vi "Common_UpdateAttributes.vi"(1 "ClassPath/LvClassRef":variant, 2 "NewAttributes":string, 3 "ClassInfo":T4[](array[typedef]), 5 "error in (no error)":errorcluster, 6 "Don't Prompt (False)":bool, 7 "Attributes":T1[](array[typedef]), 8 "Stereotype":string, 9 "Ctl-Description":string) -> (15 "CtlPath":path, 18 "Cancel":bool, 19 "error out":errorcluster)   [LabVIEW 2020] (continued)
 terminals)", "Swap Bytes", "Swap Values", "Swap Vector Element", "Swap Words", "Tab Constant", "Tab Control (classic)", "Tab Control (modern)", "Tab Control (NXG Style)", "Tab Control (system)", "Table (classic)", "Table (modern)", "Table (system)", "Tag Attribute Ring", "Tangent", "Tank (classic)", "Tank (modern)", "Target Structure", "TCP Close Connection", "TCP Create Listener", "TCP Flattened Read", "TCP Flattened Write", "TCP Flex Read", "TCP Flex Write", "TCP Network Connection Refnum", "TCP Open Connection", "TCP Read", "TCP Wait On Listener", "TCP Write", "TDMS Advanced Asynchronous Read (Data Ref)", "TDMS Advanced Asynchronous Write (Data Ref)", "TDMS Close", "TDMS Configure Asynchronous Reads (Data Ref)", "TDMS Configure Asynchronous Writes (Data Ref)", "TDMS Defragment", "TDMS Delete Data", "TDMS File", "TDMS Flush", "TDMS Get Asynchronous Read Status (Data Ref)", "TDMS Get Asynchronous Write Status (Data Ref)", "TDMS Get Properties", "TDMS In Memory Close", "TDMS In Memory Open", "TDMS In Memory Read Bytes", "TDMS List Contents", "TDMS Open", "TDMS Read", "TDMS Refnum To File ID", "TDMS Set Properties", "TDMS Write", "TDMS Write IP", "Temporary Directory", "TestSRQ", "TestSys", "Text & Pict Ring (classic)", "Text & Pict Ring (modern)", "Text Button", "Text Ring (block diagram constant)", "Text Ring (classic)", "Text Ring (modern)", "Text Ring (system)", "Text to UTF-8", "Thermometer (classic)", "Thermometer (modern)", "Threshold 1D Array", "Tick Count (ms)", "Time Stamp (block diagram constant)", "Time Stamp Control (classic)", "Time Stamp Control (modern)", "Time Stamp Control (system)", "Time Stamp Indicator (classic)", "Time Stamp Indicator (modern)", "Timed Loop", "Timed Sequence", "TLS configuration", "TLS Connection?", "To Byte Integer", "To Double Precision Complex", "To Double Precision Float", "To Extended Precision Complex", "To Extended Precision Float", "To Fixed-Point", "To Long Integer", "To Lower Case", "To More Generic Class", "To More Specific Class", "To OLE Variant", "To Probe String", "To Quad Integer", "To Single Precision Complex", "To Single Precision Float", "To Time Stamp", "To Unsigned Byte Integer", "To Unsigned Long Integer", "To Unsigned Quad Integer", "To Unsigned Word Integer", "To Upper Case", "To Variant", "To Word Integer", "Traditional DAQ Channel (block diagram constant)", "Traditional DAQ Channel (classic)", "Traditional DAQ Channel (modern)", "Transpose 1D Array", "Transpose 2D Array", "Transpose Matrix", "Tree (classic)", "Tree (modern)", "Tree (system)", "Trigger", "TriggerList", "Two Button Dialog", "Type and Creator", "Type Cast", "Type Error", "Type Must Be Array", "Type Must Be Cluster", "Type Of", "Type Specialization Structure", "UDP Close", "UDP Multicast Open", "UDP Network Connection Refnum", "UDP Open", "UDP Read", "UDP Write", "Unbitpack from Array", "Unbundle", "Unbundle By Name", "Unflatten From JSON", "Unflatten From String", "Unflatten From XML", "Unleak Variant Value Reference", "Unpackage Matrix", "Unregister For Events", "Unregister Session", "Up Arrow", "Up Bow Valve (flat)", "Up Bow Valve (outline)", "Up Bow Valve (shaded)", "Up Rect Valve (flat)", "Up Rect Valve (outline)", "Up Rect Valve (shaded)", "Up Tee (flat)", "Up Tee (shaded)", "User Defined Refnum", "User Defined Refnum Tag (block diagram constant)", "User Defined Refnum Tag (classic)", "User Defined Refnum Tag (modern)", "User Defined Refnum Tag Flatten (classic)", "User Defined Refnum Tag Flatten (modern)", "User Defined Tag (block diagram constant)", "User Defined Tag (classic)", "User Defined Tag (modern)", "User Item", "UTF-8 String To Byte Array", "UTF-8 to Text", "Variable Class Specifier Constant", "Variable Name Constant", "Variant", "Variant To Data", "Variant To Flattened String", "Vert Line", "Vert Pipe (flat)", "Vert Pipe (shaded)", "Vert Rocker", "Vertical Fill Slide (classic)", "Vertical Fill Slide (modern)", "Vertical Gradient Oval", "Vertical Gradient Rectangle", "Vertical Gradient Rounded Rectangle", "Vertical Graduated Bar", "Vertical Pointer Slide (classic)", "Vertical Pointer Slide (modern)", "Vertical Pointer Slide (system)", "Vertical Progress Bar (modern)", "Vertical Progress Bar (system)", "Vertical Scrollbar", "Vertical Slide (system)", "Vertical Slide Switch (classic)", "Vertical Slide Switch (modern)", "Vertical Smooth Box", "Vertical Splitter Bar", "Vertical Splitter Bar (Classic)", "Vertical Splitter Bar (NXG Style)", "Vertical Splitter Bar (System)", "Vertical Switch", "Vertical Toggle Switch (classic)", "Vertical Toggle Switch (modern)", "VI Library", "VI Refnum", "VI Server Reference", "VISA Assert Interrupt Signal", "VISA Assert Trigger", "VISA Assert Utility Signal", "VISA Clear", "VISA Close", "VISA Disable Event", "VISA Discard Events", "VISA Enable Event", "VISA Find Resource", "VISA Flush I/O Buffer", "VISA GPIB Command", "VISA GPIB Control ATN", "VISA GPIB Control REN", "VISA GPIB Pass Control", "VISA GPIB Send IFC", "VISA In 16", "VISA In 32", "VISA In 64", "VISA In 8", "VISA Lock", "VISA Map Address", "VISA Map Trigger", "VISA Memory Allocation", "VISA Memory Allocation Ex", "VISA Memory Free", "VISA Move", "VISA Move In 16", "VISA Move In 32", "VISA Move In 64", "VISA Move In 8", "VISA Move Out 16", "VISA Move Out 32", "VISA Move Out 64", "VISA Move Out 8", "VISA Open", "VISA Out 16", "VISA Out 32", "VISA Out 64", "VISA Out 8", "VISA Peek 16", "VISA Peek 32", "VISA Peek 64", "VISA Peek 8", "VISA Poke 16", "VISA Poke 32", "VISA Poke 64", "VISA Poke 8", "VISA Read", "VISA Read STB", "VISA Read To File", "VISA Refnum to Session", "VISA Resource Name", "VISA resource name (classic)", "VISA resource name (modern)", "VISA Set I/O Buffer Size", "VISA Status Description", "VISA Unlock", "VISA Unmap Address", "VISA Unmap Trigger", "VISA USB Control In", "VISA USB Control Out", "VISA VXI Cmd or Query", "VISA Wait on Event", "VISA Write", "VISA Write From File", "Volume Info", "Wait (ms)", "Wait For Activity", "Wait For Front Panel Activity", "Wait for GPIB RQS", "Wait on Notification", "Wait on Notification from Multiple", "Wait on Notification from Multiple with Notifier History", "Wait on Notification with Notifier History", "Wait on Occurrence", "Wait Until Next ms Multiple", "WaitSRQ", "Waveform Chart", "Waveform Chart (classic)", "Waveform Chart (modern)", "Waveform Graph (classic)", "Waveform Graph (modern)", "While Loop #1", "While Loop #2", "White Space?", "Write Datalog", "Write Device", "Write File", "Write Multiple Elements to Stream", "Write Single Element to Stream", "Write to Binary File", "Write to Text File", "Write Variable", "Write Variable with Timeout", "XY Graph (classic)", "XY Graph (modern)", "Y-th Root of X"]
                      w633 = refnum<vi> refnum  # Set
                      n218 = Format Into String(format string="Set(%s)", w622) -> (resulting string=w620:string)  [unwired: 2 in, 1 out]
                      n219 = call "Common_UpdateAttributes_DataTypeStringToEnum.vi"("Classes"=w627, "DataTypeString"=w620) -> ("Second"=w626:i32, "First(Path)"=w624:path, "First"=w625:i32)  [unwired: 4 in, 3 out]
                      n220 = New VI Object(vi object class=w633, owner refnum=w632, style=w630, position/next to=w631, 8:w634) -> (object refnum=w629:refnum<vi>, 0:w635:errorcluster)  [unwired: 3 out]
                      n221 = property class="Set"(reference=w629) -> ("SetElem"=w628:refnum<vi>)  [unwired: 1 in, 2 out]
                      n222 = Empty String/Path?(string/path=w624) -> (empty?=w623:bool)
                      n223 = case shown="True" w623 {
                        tunnel: w628 -> [w641 w645]
                        tunnel: w624 -> [_ w644]
                        tunnel: w626 -> [w639 _]
                        tunnel: w625 -> [w638 _]
                        frame True {
                          w636 = refnum<vi> refnum  # Numeric
                          n224 = invoke class="Ctl" method="Replace"(reference=w641, "Style"=w638) -> (error out=w642:errorcluster, "Replace"=w640:refnum<vi>)  [unwired: 4 in, 4 out]
                          n225 = To More Specific Class(target class=w636, reference=w640, error in=w642) -> (specific class reference=w637:refnum<vi>, error out=w643:errorcluster)
                          n226 = property class="Numeric"(reference=w637, error in=w643, "Representation"=w639) -> ()  [unwired: 2 out]
                        }
                        frame False {
                          n227 = invoke class="Ctl" method="Replace"(reference=w645, "Path"=w644) -> ()  [unwired: 4 in, 6 out]
                        }
                      }
                    }
                    frame "Map" {
                      w661 = 3488 items=[".NET Container", ".NET Refnum", "2D Picture", "3D Picture", "Absolute Value", "Accept TLS", "Access Rights", "ActiveX Container", "Add", "Add (with error terminals)", "Add Array Elements", "Add Entropy", "Add Private Key To TLS Configuration", "Add Trusted Certificate To TLS Configuration", "Agitator", "AllSpoll", "Always Copy", "And", "And Array Elements", "Append True/False String", "Application Refnum", "Array (block diagram constant)", "Array (classic)", "Array (modern)", "Array Interface Control", "Array Max & Min", "Array of Strings to Path", "Array Size", "Array Subset", "Array To Cluster", "Array To Spreadsheet String", "ArrayMemInfo", "Assert Structural Type Match", "Assert Structural Type Mismatch", "Atmospheric Tank (classic)", "Atmospheric Tank (modern)", "Automation Close", "Automation Open", "Automation Refnum", "Avogadro Constant (1/mol)", "Base 10 Logarithm Of e", "Bin #1", "Bin #2", "Bitpack to Array", "Bluetooth Close Connection", "Bluetooth Create Listener", "Bluetooth Discover", "Bluetooth Network Connection Refnum", "Bluetooth Open Connection", "Bluetooth Read", "Bluetooth Wait On Listener", "Bluetooth Write", "Boolean Array To Number", "Boolean To (0,1)", "Build Array", "Build Cluster Array", "Build Map", "Build Matrix", "Build Path", "Build Set", "Build Waveform", "Bundle", "Bundle By Name", "Byte Array To String", "Byte Array To UTF-8 String", "Byte Stream File Refnum", "Call By Reference", "Call Chain", "Call Library Function Node", "Call Parent Class Method", "CAN Channel (block diagram constant)", "CAN Channel (classic)", "CAN Channel (modern)", "CAN Channel (system)", "CAN Interface (block diagram constant)", "CAN Interface (classic)", "CAN Interface (modern)", "CAN Interface (system)", "CAN Task (block diagram constant)", "CAN Task (classic)", "CAN Task (modern)", "CAN Task (system)", "Cancel Button (modern)", "Cancel Button (system)", "Cancel Notification", "Carriage Return Constant", "Case Structure", "Cast Unit Bases", "Check Valve", "Checkbox (classic)", "CheckBox (modern)", "Checkbox (system)", "Class Specifier Constant", "Classic Color Box", "Classic Color Ramp", "Classic Horizontal Slide Switch", "Classic Vertical Slide", "Clear Fixed-Point Overflow Status", "Close File", "Close File (deprecated)", "Close Python Session", "Close Reference", "Close TLS Configuration", "Close Variable Connection", "Closure Structure", "Cluster (classic)", "Cluster (modern)", "Cluster Constant", "Cluster To Array", "Code Interface Node", "Coerce To Type", "Collection Size", "Color Box Constant", "Color Box Thin Border", "Colored Rectangle (broken?)", "Combo Box (classic)", "Combo Box (modern)", "Combo Box (system)", "Combo Box Constant", "Complex Conjugate", "Complex To Polar", "Complex To Re/Im", "Compound Arithmetic", "Compressor", "Concatenate Strings", "Conditional Disable Structure", "Constructor Node", "Control & Simulation Loop", "Control Help Window", "Control Online Help", "Control Refnum", "Convert Unit", "Conveyer", "Copy", "Copy (deprecated)", "Cosecant", "Cosine", "Cotangent", "CPU Information", "Create Folder", "Create Network Stream Endpoint", "Create Network Stream Reader Endpoint", "Create Network Stream Writer Endpoint", "Create Stream", "Create Unique Network Stream Endpoint", "Create Unique Network Stream Reader Endpoint", "Create Unique Network Stream Writer Endpoint", "Create User Event", "Current Processor ID", "Current VI's Menubar", "Current VI's Path", "DAQmx Analog Trigger Source (block diagram constant)", "DAQmx Analog Trigger Source (classic)", "DAQmx Analog Trigger Source (modern)", "DAQmx Analog Trigger Source (system)", "DAQmx Device Name (block diagram constant)", "DAQmx Device Name (classic)", "DAQmx Device Name (modern)", "DAQmx Device Name (system)", "DAQmx Global Channel (block diagram constant)", "DAQmx Global Channel (classic)", "DAQmx Global Channel (modern)", "DAQmx Global Channel (system)", "DAQmx Physical Channel (block diagram constant)", "DAQmx Physical Channel (classic)", "DAQmx Physical Channel (modern)", "DAQmx Physical Channel (system)", "DAQmx Scale Name (block diagram constant)", "DAQmx Scale Name (classic)", "DAQmx Scale Name (modern)", "DAQmx Scale Name (system)", "DAQmx Switch (block diagram constant)", "DAQmx Switch (classic)", "DAQmx Switch (modern)", "DAQmx Switch (system)", "DAQmx Task Name (block diagram constant)", "DAQmx Task Name (classic)", "DAQmx Task Name (modern)", "DAQmx Task Name (system)", "DAQmx Terminal (block diagram constant)", "DAQmx Terminal (classic)", "DAQmx Terminal (modern)", "DAQmx Terminal (system)", "Data Cache Size", "Data Log File Refnum", "Data Value Reference", "Data Value Reference Constant", "DataSocket Close", "DataSocket Open", "DataSocket Read", "DataSocket Refnum", "DataSocket Write", "Date/Time To Seconds", "Decimal Digit?", "Decimal String To Number", "Decimate 1D Array", "DecomposeLockDataValRef", "DecomposeVariant", "Decrement", "Default Directory", "Delete", "Delete (deprecated)", "Delete Data Value Reference", "Delete From Array", "Delete Menu Items", "Delete Variant Attribute", "Delete Waveform Attribute", "Deny Access", "Dequeue Element", "Destroy Stream Endpoint", "Destroy User Event", "DevClear", "DevClearList", "Device Control/Status", "Device Refnum", "Diagram Disable Structure", "Dial (classic)", "Dial (modern)", "Digital Data (classic)", "Digital Data (modern)", "Digital Waveform Graph (classic)", "Digital Waveform Graph (modern)", "Direct Variable Read", "Direct Variable Write", "Divide", "Divide (with error terminals)", "Dlg Horiz Scrollbar", "Dlg Mac Group Box", "Dlg Numeric #1", "Dlg Numeric #2", "Dlg String", "Dlg Vert Scrollbar", "Down Arrow", "Down Bow Valve (flat)", "Down Bow Valve (outline)", "Down Bow Valve (shaded)", "Down Rect Valve (flat)", "Down Rect Valve (outline)", "Down Rect Valve (shaded)", "Down Tee (flat)", "Down Tee (shaded)", "Dynamic FPGA Interface Cast", "Eased Corner Rectangle", "Element of Set?", "Elementary Charge (C)", "Empty Array?", "Empty Collection?", "Empty Path Constant", "Empty String Constant", "Empty String/Path?", "Enable Menu Tracking", "EnableLocal", "EnableRemote", "End of Line Constant", "Enqueue Element", "Enqueue Element At Opposite End", "Enum (classic)", "Enum (modern)", "Enum (system)", "Enum Constant", "EOF", "Equal To 0?", "Equal?", "Error Ring Constant", "Event Callback Refnum", "Event Data Node", "Event Structure", "Exchanger", "Exclusive Or", "Exponential", "Exponential (Arg) -1", "Expression Node", "False Constant", "Feedback Node", "FieldPoint IO Point (block diagram constant)", "FieldPoint IO Point (classic)", "FieldPoint IO Point (modern)", "FIFO Refnum", "File Dialog", "File Dialog (deprecated)", "File Path Control (classic)", "File Path Control (modern)", "File Path Control (system)", "File Path Indicator (classic)", "File Path Indicator (modern)", "File/Directory Info", "File/Directory Info (deprecated)", "FindLstn", "FindRQS", "First Call?", "Fixed-Point Overflow?", "Fixed-Point to Integer Cast", "Flat Box", "Flat Circle", "Flat Down Triangle", "Flat Frame", "Flat Left Triangle", "Flat Right Triangle", "Flat Round Button", "Flat Rounded Box", "Flat Sequence Structure", "Flat Square Button", "Flat Up Triangle", "Flatten To JSON", "Flatten To String", "Flatten To XML", "Flattened String To Variant", "Floating Point Equal?", "Flush Event Queue", "Flush File", "Flush File (deprecated)", "Flush Queue", "Flush Stream", "For Loop", "Fork", "Format Date/Time String", "Format Into File", "Format Into String", "Format Value", "Formula Node", "FPGA Refnum to Session", "Fract/Exp String To Number", "Framed Color Box (classic)", "Framed Color Box (modern)", "Free Label", "Furnace", "Gauge (classic)", "Gauge (modern)", "Gauge for Simon", "Generate Front Panel Activity", "Generate Occurrence", "Generate User Event", "Generate User-Defined Trace Event", "Get Control Values by Index", "Get Datalog Position", "Get Date/Time In Seconds", "Get Date/Time String", "Get Drag Drop Data", "Get File Position", "Get File Size", "Get Fixed-Point Components", "Get Help Window Status", "Get Matrix Diagonal", "Get Matrix Elements", "Get Menu Item Info", "Get Menu Selection", "Get Menu Short Cut Info", "Get Notifier Status", "Get Number of Records", "Get Permissions", "Get Queue Status", "Get Submatrix", "Get Type and Creator", "Get Variant Attribute", "Get Volume Info", "Get Waveform Attribute", "Get Waveform Components", "Global Variable", "GPIB Clear", "GPIB Initialization", "GPIB Misc", "GPIB Read", "GPIB Serial Poll", "GPIB Status", "GPIB Trigger", "GPIB Wait", "GPIB Write", "Gravitational Constant (N m2/kg2)", "Greater Or Equal To 0?", "Greater Or Equal?", "Greater Than 0?", "Greater?", "Handle Peek", "Handle Poke", "Hex Digit?", "Hexadecimal String To Number", "Hopper #1", "Hopper #2", "Horiz Line", "Horiz Pipe (flat)", "Horiz Pipe (shaded)", "Horizontal Button Box", "Horizontal Fill Slide (classic)", "Horizontal Fill Slide (modern)", "Horizontal Gradient Oval", "Horizontal Gradient Rectangle", "Horizontal Gradient Rounded Rectangle", "Horizontal Graduated Bar", "Horizontal Pointer Slide (classic)", "Horizontal Pointer Slide (modern)", "Horizontal Pointer Slide (system)", "Horizontal Progress Bar (modern)", "Horizontal Progress Bar (system)", "Horizontal Scrollbar", "Horizontal Slide (classic)", "Horizontal Slide (system)", "Horizontal Smooth Box", "Horizontal Splitter Bar", "Horizontal Splitter Bar (Classic)", "Horizontal Splitter Bar (NXG Style)", "Horizontal Splitter Bar (System)", "Horizontal Switch", "Horizontal Tank", "Horizontal Toggle Switch (classic)", "Horizontal Toggle Switch (modern)", "Hyperbolic Cosecant", "Hyperbolic Cosine", "Hyperbolic Cotangent", "Hyperbolic Secant", "Hyperbolic Sine", "Hyperbolic Tangent", "IMAQ Session", "Implies", "In Place Element Structure", "In Range and Coerce", "Include Fixed-Point Overflow Status", "Increment", "Index & Bundle Cluster Array", "Index Array", "Index String Array", "Initialize Array", "Inline C Node", "Insert Into Array", "Insert Into Map", "Insert Into Set", "Insert Menu Items", "Integer to Fixed-Point Cast", "Intensity Chart (classic)", "Intensity Chart (modern)", "Intensity Graph (classic)", "Intensity Graph (modern)", "Interleave 1D Arrays", "Interpolate 1D Array", "Inverse Cosecant", "Inverse Cosine", "Inverse Cotangent", "Inverse Hyperbolic Cosecant", "Inverse Hyperbolic Cosine", "Inverse Hyperbolic Cotangent", "Inverse Hyperbolic Secant", "Inverse Hyperbolic Sine", "Inverse Hyperbolic Tangent", "Inverse Secant", "Inverse Sine", "Inverse Tangent", "Inverse Tangent (2 Input)", "Invoke Node", "IP To String", "IrDA Close Connection", "IrDA Create Listener", "IrDA Discover", "IrDA Network Connection Refnum", "IrDA Open Connection", "IrDA Read", "IrDA Wait On Listener", "IrDA Write", "IsDebuggingActive", "IVI Delete Session", "IVI Logical Name (block diagram constant)", "IVI Logical Name (classic)", "IVI Logical Name (modern)", "IVI New Session", "Join", "Join Numbers", "Junction", "Knob (classic)", "Knob (modern)", "Label (modern)", "Label (system)", "Labeled Oblong Button", "Labeled Rectangular Button", "Labeled Round Button", "Labeled Square Button", "LabVIEW Object", "Leak Variant Value Reference", "LED Button", "Left Arrow", "Left Bow Valve (flat)", "Left Bow Valve (outline)", "Left Bow Valve (shaded)", "Left Down Elbow (flat)", "Left Down Elbow (shaded)", "Left Pump (flat)", "Left Pump (shaded)", "Left Rect Valve (flat)", "Left Rect Valve (outline)", "Left Rect Valve (shaded)", "Left Tee (flat)", "Left Tee (shaded)", "Left Up Elbow (flat)", "Left Up Elbow (shaded)", "Less Or Equal To 0?", "Less Or Equal?", "Less Than 0?", "Less?", "Lexical Class", "Line (chiseled, system)", "Line (chiseled, thick)", "Line (chiseled, thin)", "Line (thick)", "Line (thin)", "Line Feed Constant", "Line with Arrow (thick)", "Line with Arrow (thin)", "List Directory", "List Folder", "Listbox (classic)", "Listbox (modern)", "Listbox (system)", "Listbox Symbol Ring Constant", "Load Certificates Into Memory", "Load Private Key Into Memory", "Local Variable", "Lock Range", "Logarithm Base 10", "Logarithm Base 2", "Logarithm Base X", "Logical Shift", "Look In Map", "Lookup Channel Probe", "Lossy Enqueue Element", "Lowered Box (thick)", "Lowered Rounded Box", "Machine Epsilon", "Make TLS Configuration Immutable", "MakeAddr", "Mantissa & Exponent", "Map", "Map Constant", "Match First String", "Match Pattern", "Match True/False String", "MathScript Call By Reference", "MathScript Node", "MATLAB script", "Matrix Size", "Max & Min", "Menu Refnum", "Menu Ring (classic)", "Menu Ring (modern)", "Menu-Popup Ring", "Merge Errors", "Merge Signals", "Meter (classic)", "Meter (modern)", "Mixed Checkbox (system)", "Mixed Signal Graph", "Molar Gas Constant (J/(mol K))", "Motion Resource (block diagram constant)", "Motion Resource (classic)", "Motion Resource (modern)", "Motor (flat)", "Motor (shaded)", "Move", "Move (deprecated)", "Multi-Segment Pipe", "Multicolumn Listbox (classic)", "Multicolumn Listbox (modern)", "Multicolumn Listbox (system)", "Multiply", "Multiply (with error terminals)", "Multiply Array Elements", "Multirate Structure", "Natural Logarithm", "Natural Logarithm (Arg +1)", "Natural Logarithm Base", "Natural Logarithm Of 10", "Natural Logarithm Of 2", "Natural Logarithm Of Pi", "Negate", "Negative Infinity", "New Data Value Reference", "New Directory", "New File", "New TLS Configuration", "New VI", "New VI Object", "Not", "Not A Number/Path/Refnum?", "Not A Path Constant", "Not a Refnum Constant", "Not a Shared Variable", "Not And", "Not Equal To 0?", "Not Equal?", "Not Exclusive Or", "Not Or", "Notifier Refnum", "Number of Cache Levels", "Number To Boolean Array", "Number To Decimal String", "Number To Engineering String", "Number To Exponential String", "Number To Fractional String", "Number To Hexadecimal String", "Number To Octal String", "Numeric Constant", "Numeric Control (classic)", "Numeric Control (modern)", "Numeric Control (system)", "Numeric Indicator (classic)", "Numeric Indicator (modern)", "Obtain Notifier", "Obtain Queue", "Occurrence Refnum", "Octal Digit?", "Octal String To Number", "OK Button (modern)", "OK Button (system)", "Old VISA Open", "OLE Variant", "One Button Dialog", "Open and Verify Variable Connection", "Open Application Reference", "Open Device", "Open Dynamic Bitfile Reference", "Open File", "Open Python Session", "Open Tank (flat classic)", "Open Tank (shaded classic)", "Open Variable Connection", "Open Variable Connection in Background", "Open VI Object Reference", "Open VI Reference", "Open/Create/Replace Datalog", "Open/Create/Replace File", "Or", "Or Array Elements", "Oval with Shadow", "Package Matrix", "PassControl", "Path Constant", "Path to Array of Strings", "Path To String", "Path Type", "Pi", "Pi Divided By 2", "Pi Multiplied By 2", "Pick Line", "Pict Ring (classic)", "Pict Ring (modern)", "Pict Ring (system)", "PixMap", "PixMap (warning: dangerous)", "Planck's Constant (J/Hz)", "Platform Flat Square Button", "Plug-In Control", "Polar To Complex", "Polar To Re/Im", "Positive Infinity", "Power Of 10", "Power Of 2", "Power Of X", "PPoll", "PPollConfig", "PPollUnconfig", "Preallocated Read from Binary File", "Preserve Run-Time Class", "Pressure Tank (flat)", "Pressure Tank (shaded)", "Preview Queue Element", "Printable?", "Property Node", "Pulldown Menu Ring", "Push Button", "Python Node", "Python Session Refnum", "Queue Refnum", "Quit LabVIEW", "Quotient & Remainder", "Race Structure", "Radio Button (system)", "Radio Buttons (classic)", "Radio Buttons (modern)", "Radio Buttons (system)", "Raised Box (classic)", "Raised Box (modern)", "Raised Circle", "Raised Down Triangle", "Raised Frame", "Raised Left Triangle", "Raised Right Triangle", "Raised Rounded Box", "Raised Up Triangle", "Random Number (0-1)", "RcvRespMsg", "Re-accept TLS", "Re/Im To Complex", "Re/Im To Polar", "Read Datalog", "Read Device", "Read File", "Read from Binary File", "Read from Text File", "Read Map Max & Min Keys", "Read Multiple Elements from Stream", "Read Set Max & Min", "Read Single Element from Stream", "Read Variable", "Read Variable with Timeout", "ReadStatus", "Receive", "ReceiveSetup", "Recessed Box", "Recessed Circle", "Recessed Down Triangle", "Recessed Frame (modern)", "Recessed Frame (system)", "Recessed Left Triangle", "Recessed Menu Ring", "Recessed Right Triangle", "Recessed Rounded Box", "Recessed Up Triangle", "Reciprocal", "Reciprocal Of e", "Reciprocal Of Pi", "RecomposeUnlockDataValRef (warning: dangerous)", "RecomposeVariant (warning: dangerous)", "Rectangular Stop Button", "Refnum to Path", "Refnum to Session", "Region", "Register Event Callback", "Register For Events", "Register Session", "Release Notifier", "Release Queue", "Remove Fixed-Point Overflow Status", "Remove From Map", "Remove From Set", "Replace Array Subset", "Replace Substring", "Request Deallocation", "ResetSys", "Reshape Array", "Resize Matrix", "Resource Index", "Reverse 1D Array", "Reverse String", "Right Arrow", "Right Bow Valve (flat)", "Right Bow Valve (outline)", "Right Bow Valve (shaded)", "Right Down Elbow (flat)", "Right Down Elbow (shaded)", "Right Pump (flat)", "Right Pump (shaded)", "Right Rect Valve (flat)", "Right Rect Valve (outline)", "Right Rect Valve (shaded)", "Right Tee (flat)", "Right Tee (shaded)", "Right Up Elbow (flat)", "Right Up Elbow (shaded)", "Rocker", "Rotary Feeder", "Rotate", "Rotate 1D Array", "Rotate Left With Carry", "Rotate Right With Carry", "Rotate String", "Round Button", "Round LED (classic)", "Round LED (modern)", "Round Light", "Round Push Button", "Round Push Button (profile)", "Round Radio Button", "Round Stop Button", "Round To Nearest", "Round Toward +Infinity", "Round Toward -Infinity", "Rounded Rectangle with Shadow", "RT FIFO Create", "RT FIFO Delete", "RT FIFO Read", "RT FIFO Write", "Rydberg Constant (1/m)", "Scale By Power Of 2", "Scan From File", "Scan From String", "Scan String For Tokens", "Scan Value", "Scanned Variable Read", "Scanned Variable Write", "Search 1D Array", "Search and Replace String", "Search Variable Container", "Search/Split String", "Secant", "Seconds To Date/Time", "Seek", "Select", "Send", "Send Notification", "SendCmds", "SendDataBytes", "SendIFC", "SendList", "SendLLO", "SendSetup", "Session to Refnum", "Set", "Set Constant", "Set Control Values by Index", "Set Datalog Position", "Set File Position", "Set File Size", "Set Matrix Diagonal", "Set Matrix Elements", "Set Menu Item Info", "Set Number of Records", "Set Occurrence", "Set Permissions", "Set Submatrix", "Set Type and Creator", "Set Variant Attribute", "Set Waveform Attribute", "SetRWLS", "SetTimeOut", "Shared Variable", "Shared Variable Constant", "Shared Variable Control (classic)", "Shared Variable Control (modern)", "Shared Variable to String", "Sign", "Simple Horizontal Slide", "Simple Numeric", "Simple String", "Simple Vertical Slide", "Sinc", "Sine", "Sine & Cosine", "Size Handle", "Slide Switch", "Smoothed Oval", "Smoothed Rounded Rectangle", "Sort 1D Array", "Sort Array of String", "Speed Of Light In Vacuum (m/sec)", "Spin Control (system)", "Split 1D Array", "Split Button", "Split Number", "Split Signals", "Spreadsheet String To Array", "Square", "Square Button", "Square LED (classic)", "Square LED (modern)", "Square Light", "Square Push Button", "Square Push Button (profile)", "Square Radio Button", "Square Root", "Stacked Sequence Structure", "Start TLS", "State", "State Diagram", "Static VI Reference", "Stop", "Stop Button", "String Constant", "String Control (classic)", "String Control (modern)", "String Control (system)", "String Indicator (classic)", "String Indicator (modern)", "String Length", "String Subset", "String To Byte Array", "String To IP", "String To Path", "String to Shared Variable", "Strip Path", "SubPanel", "SubPanel (Classic)", "SubPanel (NXG Style)", "SubPanel (System)", "Subtract", "Subtract (with error terminals)", "Swap Bytes", "Swap Values", "Swap Vector Element", "Swap Words", "Tab Constant", "Tab Control (classic)", "Tab Control (modern)", "Tab Control (NXG Style)", "Tab Control (system)", "Table (classic)", "Table (modern)", "Table (system)", "Tag Attribute Ring", "Tangent", "Tank (classic)", "Tank (modern)", "Target Structure", "TCP Close Connection", "TCP Create Listener", "TCP Flattened Read", "TCP Flattened Write", "TCP Flex Read", "TCP Flex Write", "TCP Network Connection Refnum", "TCP Open Connection", "TCP Read", "TCP Wait On Listener", "TCP Write", "TDMS Advanced Asynchronous Read (Data Ref)", "TDMS Advanced Asynchronous Write (Data Ref)", "TDMS Close", "TDMS Configure Asynchronous Reads (Data Ref)", "TDMS Configure Asynchronous Writes (Data Ref)", "TDMS Defragment", "TDMS Delete Data", "TDMS File", "TDMS Flush", "TDMS Get Asynchronous Read Status (Data Ref)", "TDMS Get Asynchronous Write Status (Data Ref)", "TDMS Get Properties", "TDMS In Memory Close", "TDMS In Memory Open", "TDMS In Memory Read Bytes", "TDMS List Contents", "TDMS Open", "TDMS Read", "TDMS Refnum To File ID", "TDMS Set Properties", "TDMS Write", "TDMS Write IP", "Temporary Directory", "TestSRQ", "TestSys", "Text & Pict Ring (classic)", "Text & Pict Ring (modern)", "Text Button", "Text Ring (block diagram constant)", "Text Ring (classic)", "Text Ring (modern)", "Text Ring (system)", "Text to UTF-8", "Thermometer (classic)", "Thermometer (modern)", "Threshold 1D Array", "Tick Count (ms)", "Time Stamp (block diagram constant)", "Time Stamp Control (classic)", "Time Stamp Control (modern)", "Time Stamp Control (system)", "Time Stamp Indicator (classic)", "Time Stamp Indicator (modern)", "Timed Loop", "Timed Sequence", "TLS configuration", "TLS Connection?", "To Byte Integer", "To Double Precision Complex", "To Double Precision Float", "To Extended Precision Complex", "To Extended Precision Float", "To Fixed-Point", "To Long Integer", "To Lower Case", "To More Generic Class", "To More Specific Class", "To OLE Variant", "To Probe String", "To Quad Integer", "To Single Precision Complex", "To Single Precision Float", "To Time Stamp", "To Unsigned Byte Integer", "To Unsigned Long Integer", "To Unsigned Quad Integer", "To Unsigned Word Integer", "To Upper Case", "To Variant", "To Word Integer", "Traditional DAQ Channel (block diagram constant)", "Traditional DAQ Channel (classic)", "Traditional DAQ Channel (modern)", "Transpose 1D Array", "Transpose 2D Array", "Transpose Matrix", "Tree (classic)", "Tree (modern)", "Tree (system)", "Trigger", "TriggerList", "Two Button Dialog", "Type and Creator", "Type Cast", "Type Error", "Type Must Be Array", "Type Must Be Cluster", "Type Of", "Type Specialization Structure", "UDP Close", "UDP Multicast Open", "UDP Network Connection Refnum", "UDP Open", "UDP Read", "UDP Write", "Unbitpack from Array", "Unbundle", "Unbundle By Name", "Unflatten From JSON", "Unflatten From String", "Unflatten From XML", "Unleak Variant Value Reference", "Unpackage Matrix", "Unregister For Events", "Unregister Session", "Up Arrow", "Up Bow Valve (flat)", "Up Bow Valve (outline)", "Up Bow Valve (shaded)", "Up Rect Valve (flat)", "Up Rect Valve (outline)", "Up Rect Valve (shaded)", "Up Tee (flat)", "Up Tee (shaded)", "User Defined Refnum", "User Defined Refnum Tag (block diagram constant)", "User Defined Refnum Tag (classic)", "User Defined Refnum Tag (modern)", "User Defined Refnum Tag Flatten (classic)", "User Defined Refnum Tag Flatten (modern)", "User Defined Tag (block diagram constant)", "User Defined Tag (classic)", "User Defined Tag (modern)", "User Item", "UTF-8 String To Byte Array", "UTF-8 to Text", "Variable Class Specifier Constant", "Variable Name Constant", "Variant", "Variant To Data", "Variant To Flattened String", "Vert Line", "Vert Pipe (flat)", "Vert Pipe (shaded)", "Vert Rocker", "Vertical Fill Slide (classic)", "Vertical Fill Slide (modern)", "Vertical Gradient Oval", "Vertical Gradient Rectangle", "Vertical Gradient Rounded Rectangle", "Vertical Graduated Bar", "Vertical Pointer Slide (classic)", "Vertical Pointer Slide (modern)", "Vertical Pointer Slide (system)", "Vertical Progress Bar (modern)", "Vertical Progress Bar (system)", "Vertical Scrollbar", "Vertical Slide (system)", "Vertical Slide Switch (classic)", "Vertical Slide Switch (modern)", "Vertical Smooth Box", "Vertical Splitter Bar", "Vertical Splitter Bar (Classic)", "Vertical Splitter Bar (NXG Style)", "Vertical Splitter Bar (System)", "Vertical Switch", "Vertical Toggle Switch (classic)", "Vertical Toggle Switch (modern)", "VI Library", "VI Refnum", "VI Server Reference", "VISA Assert Interrupt Signal", "VISA Assert Trigger", "VISA Assert Utility Signal", "VISA Clear", "VISA Close", "VISA Disable Event", "VISA Discard Events", "VISA Enable Event", "VISA Find Resource", "VISA Flush I/O Buffer", "VISA GPIB Command", "VISA GPIB Control ATN", "VISA GPIB Control REN", "VISA GPIB Pass Control", "VISA GPIB Send IFC", "VISA In 16", "VISA In 32", "VISA In 64", "VISA In 8", "VISA Lock", "VISA Map Address", "VISA Map Trigger", "VISA Memory Allocation", "VISA Memory Allocation Ex", "VISA Memory Free", "VISA Move", "VISA Move In 16", "VISA Move In 32", "VISA Move In 64", "VISA Move In 8", "VISA Move Out 16", "VISA Move Out 32", "VISA Move Out 64", "VISA Move Out 8", "VISA Open", "VISA Out 16", "VISA Out 32", "VISA Out 64", "VISA Out 8", "VISA Peek 16", "VISA Peek 32", "VISA Peek 64", "VISA Peek 8", "VISA Poke 16", "VISA Poke 32", "VISA Poke 64", "VISA Poke 8", "VISA Read", "VISA Read STB", "VISA Read To File", "VISA Refnum to Session", "VISA Resource Name", "VISA resource name (classic)", "VISA resource name (modern)", "VISA Set I/O Buffer Size", "VISA Status Description", "VISA Unlock", "VISA Unmap Address", "VISA Unmap Trigger", "VISA USB Control In", "VISA USB Control Out", "VISA VXI Cmd or Query", "VISA Wait on Event", "VISA Write", "VISA Write From File", "Volume Info", "Wait (ms)", "Wait For Activity", "Wait For Front Panel Activity", "Wait for GPIB RQS", "Wait on Notification", "Wait on Notification from Multiple", "Wait on Notification from Multiple with Notifier History", "Wait on Notification with Notifier History", "Wait on Occurrence", "Wait Until Next ms Multiple", "WaitSRQ", "Waveform Chart", "Waveform Chart (classic)", "Waveform Chart (modern)", "Waveform Graph (classic)", "Waveform Graph (modern)", "While Loop #1", "While Loop #2", "White Space?", "Write Datalog", "Write Device", "Write File", "Write Multiple Elements to Stream", "Write Single Element to Stream", "Write to Binary File", "Write to Text File", "Write Variable", "Write Variable with Timeout", "XY Graph (classic)", "XY Graph (modern)", "Y-th Root of X"]
                      w664 = refnum<vi> refnum  # Map
                      n228 = Format Into String(format string="Map(%s)", w646) -> (resulting string=w647:string)  [unwired: 2 in, 1 out]
                      n229 = call "Common_UpdateAttributes_DataTypeStringToEnum.vi"("Classes"=w660, "DataTypeString"=w647) -> ("Second(Path)"=w652:path, "Second"=w651:i32, "First(Path)"=w656:path, "First"=w655:i32, "Second(Representation)"=w653:T7, "First(Representation)"=w654:T7)  [unwired: 4 in]
                      n230 = New VI Object(vi object class=w664, owner refnum=w663, style=w661, position/next to=w662, 8:w665) -> (object refnum=w659:refnum<vi>, 0:w666:errorcluster)  [unwired: 3 out]
                      n231 = property class="Map"(reference=w659) -> ("MapKey"=w650:refnum<vi>, "MapValue"=w649:refnum<vi>)  [unwired: 1 in, 2 out]
                      n232 = Empty String/Path?(string/path=w656) -> (empty?=w657:bool)
                      n233 = Empty String/Path?(string/path=w652) -> (empty?=w658:bool)
                      n234 = case shown="True" w657 {
                        tunnel: w656 -> [_ w686]
                        tunnel: w654 -> [w681 _]
                        tunnel: w655 -> [w680 _]
                        tunnel: w650 -> [w677 w685]
                        frame True {
                          w678 = refnum<vi> refnum  # Numeric
                          n235 = invoke class="Ctl" method="Replace"(reference=w677, "Style"=w680) -> (error out=w683:errorcluster, "Replace"=w682:refnum<vi>)  [unwired: 4 in, 4 out]
                          n236 = To More Specific Class(target class=w678, reference=w682, error in=w683) -> (specific class reference=w679:refnum<vi>, error out=w684:errorcluster)
                          n237 = property class="Numeric"(reference=w679, error in=w684, "Representation"=w681) -> ()  [unwired: 2 out]
                        }
                        frame False {
                          n238 = invoke class="Ctl" method="Replace"(reference=w685, "Path"=w686) -> ()  [unwired: 4 in, 6 out]
                        }
                      }
                      n239 = case shown="True" w658 {
                        tunnel: w652 -> [_ w676]
                        tunnel: w653 -> [w671 _]
                        tunnel: w651 -> [w670 _]
                        tunnel: w649 -> [w667 w675]
                        frame True {
                          w668 = refnum<vi> refnum  # Numeric
                          n240 = invoke class="Ctl" method="Replace"(reference=w667, "Style"=w670) -> (error out=w673:errorcluster, "Replace"=w672:refnum<vi>)  [unwired: 4 in, 4 out]
                          n241 = To More Specific Class(target class=w668, reference=w672, error in=w673) -> (specific class reference=w669:refnum<vi>, error out=w674:errorcluster)
                          n242 = property class="Numeric"(reference=w669, error in=w674, "Representation"=w671) -> ()  [unwired: 2 out]
                        }
                        frame False {
                          n243 = invoke class="Ctl" method="Replace"(reference=w675, "Path"=w676) -> ()  [unwired: 4 in, 6 out]
                        }
                      }
                    }
                    frame "PATH" {
                      w692 = refnum<vi> refnum  # Path
                      w693 = 3203 items=[".NET Refnum", "Absolute Value", "Access Rights", "ActiveX Container", "Add", "Add Array Elements", "Agitator", "AllSpoll", "And", "And Array Elements", "Append True/False String", "Application Refnum", "Array", "Array 1", "Array Constant", "Array Max & Min", "Array Size", "Array Subset", "Array To Cluster", "Array To Spreadsheet String", "Array of Strings to Path", "Atmospheric Tank", "Atmospheric Tank 1", "Automation Close", "Automation Open", "Automation Refnum", "Avogadro Constant (1/mol)", "Base 10 Logarithm Of e", "Bin", "Bin 1", "Bluetooth Close Connection", "Bluetooth Create Listener", "Bluetooth Discover", "Bluetooth Network Connection Refnum", "Bluetooth Open Connection", "Bluetooth Read", "Bluetooth Wait On Listener", "Bluetooth Write", "Boolean Array To Number", "Boolean To (0,1)", "Build Array", "Build Cluster Array", "Build Path", "Build Waveform", "Bundle", "Bundle By Name", "Byte Array To String", "Byte Stream File Refnum", "Call By Reference Node", "Call Chain", "Call Library Function Node", "Cancel Button", "Cancel Button 1", "Cancel Notification", "Carriage Return Constant", "Case Structure", "Cast Unit Bases", "Check Valve", "Checkbox", "Class Specifier Constant", "Classic Radio Buttons", "Close File", "Close Reference", "Cluster", "Cluster 1", "Cluster Constant", "Cluster To Array", "Code Interface Node", "Color Box", "Color Box Constant", "Color Box Thin Border", "Color Ramp", "Combo Box", "Combo Box 1", "Combo Box Constant", "Complex Conjugate", "Complex To Polar", "Complex To Re/Im", "Compound Arithmetic", "Compressor", "Concatenate Strings", "Conditional Disable Structure", "Constructor Node", "Control Help Window", "Control Online Help", "Control Refnum", "Convert Unit", "Conveyer", "Copy", "Cosecant", "Cosine", "Cotangent", "Create User Event", "Current VI's Menubar", "Current VI's Path", "DAQmx Analog Trigger Source", "DAQmx Analog Trigger Source 1", "DAQmx Analog Trigger Source 2", "DAQmx Analog Trigger Source Constant", "DAQmx Device Name", "DAQmx Device Name 1", "DAQmx Device Name 2", "DAQmx Device Name Constant", "DAQmx Global Channel", "DAQmx Global Channel 1", "DAQmx Global Channel 2", "DAQmx Global Channel Constant", "DAQmx Physical Channel", "DAQmx Physical Channel 1", "DAQmx Physical Channel 2", "DAQmx Physical Channel Constant", "DAQmx Scale Name", "DAQmx Scale Name 1", "DAQmx Scale Name 2", "DAQmx Scale Name Constant", "DAQmx Switch", "DAQmx Switch 1", "DAQmx Switch 2", "DAQmx Switch Constant", "DAQmx Task Name", "DAQmx Task Name 1", "DAQmx Task Name 2", "DAQmx Task Name Constant", "DAQmx Terminal", "DAQmx Terminal 1", "DAQmx Terminal 2", "DAQmx Terminal Constant", "Data Log File Refnum", "DataSocket Close", "DataSocket Open", "DataSocket Read", "DataSocket Refnum", "DataSocket Write", "Database Variant To Data", "Date/Time To Seconds", "Decimal Digit?", "Decimal String To Number", "Decimate 1D Array", "Decrement", "Default Directory", "Delete", "Delete From Array", "Delete Menu Items", "Delete Variant Attribute", "Delete Waveform Attribute", "Dequeue Element", "Destroy User Event", "DevClear", "DevClearList", "Device Control/Status", "Device Refnum", "Diagram Disable Structure", "Dial", "Dial 1", "Dialog Button", "Dialog Checkbox", "Dialog Chiseled Line", "Dialog Colored Rectangle", "Dialog Combo Box", "Dialog Horizontal Pointer Slide", "Dialog Horizontal Progress Bar", "Dialog Horizontal Slide", "Dialog Label", "Dialog Listbox", "Dialog Listbox 1", "Dialog Multicolumn Listbox", "Dialog Multiple Selection Multicolumn Listbox", "Dialog Numeric", "Dialog Path Control", "Dialog Pict Ring", "Dialog Radio Button", "Dialog Radio Buttons", "Dialog Recessed Frame", "Dialog Ring", "Dialog Spin Control", "Dialog String", "Dialog Tab Control", "Dialog Table", "Dialog Tree", "Dialog Vertical Pointer Slide", "Dialog Vertical Progress Bar", "Dialog Vertical Slide", "Digital Data", "Digital Data 1", "Digital Waveform Graph", "Digital Waveform Graph 1", "Digital Waveform Graph 2", "Divide", "Dlg CheckBox", "Dlg Horiz Scrollbar", "Dlg Numeric", "Dlg Numeric 2", "Dlg String", "Dlg Vert Scrollbar", "Down Arrow", "Down Bow Valve", "Down Bow Valve 1", "Down Bow Valve 2", "Down Rect Valve", "Down Rect Valve 1", "Down Rect Valve 2", "Down Tee", "Down Tee 1", "EOF", "Elementary Charge (C)", "Empty Path Constant", "Empty String Constant", "Empty String/Path?", "Enable Menu Tracking", "EnableLocal", "EnableRemote", "End of Line Constant", "Enqueue Element", "Enqueue Element At Opposite End", "Enum", "Enum 1", "Enum Constant", "Equal To 0?", "Equal?", "Error Ring Constant", "Event Callback Refnum", "Event Structure", "Exchanger", "Exclusive Or", "Exponential", "Exponential (Arg) -1", "Expression Node", "False Constant", "Feedback Node", "FieldPoint IO Point", "FieldPoint IO Point 1", "FieldPoint IO Point Constant", "File Dialog", "File Path Control", "File Path Control 1", "File Path Indicator", "File Path Indicator 1", "File/Directory Info", "FindLstn", "FindRQS", "First Call?", "Flat Box", "Flat Circle", "Flat Down Triangle", "Flat Frame", "Flat Left Triangle", "Flat Right Triangle", "Flat Round Button", "Flat Rounded Box", "Flat Sequence Structure", "Flat Square Button", "Flat Up Triangle", "Flatten To String", "Flatten To XML", "Flattened String To Variant", "Flush File", "Flush Queue", "For Loop", "Format Date/Time String", "Format Into File", "Format Into String", "Format Value", "Formula Node", "Fract/Exp String To Number", "Framed Color Box", "Framed Color Box 1", "Free Label", "Furnace", "GPIB Clear", "GPIB Initialization", "GPIB Misc", "GPIB Read", "GPIB Serial Poll", "GPIB Status", "GPIB Trigger", "GPIB Wait", "GPIB Write", "Gauge", "Gauge 1", "Generate Front Panel Activity", "Generate Occurrence", "Generate User Event", "Generic Refnum", "Generic Refnum By Reference Flatten", "Generic Refnum Deep Copy", "Generic Refnum Name", "Generic Refnum Tag", "Generic Refnum Tag By Reference Flatten", "Generic Refnum Tag Flatten", "Get Date/Time In Seconds", "Get Date/Time String", "Get Help Window Status", "Get Menu Item Info", "Get Menu Selection", "Get Menu Short Cut Info", "Get Notifier Status", "Get Queue Status", "Get Variant Attribute", "Get Waveform Attribute", "Get Waveform Components", "Global Variable", "Gravitational Constant (N m2/kg2)", "Greater Or Equal To 0?", "Greater Or Equal?", "Greater Than 0?", "Greater?", "Handle Peek", "Handle Poke", "Hex Digit?", "Hexadecimal String To Number", "HiQ-Script", "Hopper", "Hopper 1", "Horiz Line", "Horiz Pipe", "Horiz Pipe 1", "Horizontal Button Box", "Horizontal Fill Slide", "Horizontal Fill Slide 1", "Horizontal Graduated Bar", "Horizontal Pointer Slide", "Horizontal Pointer Slide 1", "Horizontal Progress Bar", "Horizontal Slide", "Horizontal Slide Switch", "Horizontal Smooth Box", "Horizontal Switch", "Horizontal Tank", "Horizontal Toggle Switch", "Horizontal Toggle Switch 1", "Hyperbolic Cosine", "Hyperbolic Sine", "Hyperbolic Tangent", "IMAQ Session", "IP To String", "IVI Delete Session", "IVI Logical Name", "IVI Logical Name 1", "IVI Logical Name Constant", "IVI New Session", "Implies", "In Range and Coerce", "Increment", "Index & Bundle Cluster Array", "Index Array", "Index String Array", "Initialize Array", "Insert Into Array", "Insert Menu Items", "Intensity Chart", "Intensity Chart 1", "Intensity Graph", "Intensity Graph 1", "Interleave 1D Arrays", "Interpolate 1D Array", "Inverse Cosine", "Inverse Hyperbolic Cosine", "Inverse Hyperbolic Sine", "Inverse Hyperbolic Tangent", "Inverse Sine", "Inverse Tangent", "Inverse Tangent (2 Input)", "Invoke Node", "IrDA Close Connection", "IrDA Create Listener", "IrDA Discover", "IrDA Network Connection Refnum", "IrDA Open Connection", "IrDA Read", "IrDA Wait On Listener", "IrDA Write", "Join Numbers", "Knob", "Knob 1", "LED Button", "Label", "Labeled Oblong Button", "Labeled Rectangular Button", "Labeled Round Button", "Labeled Square Button", "Left Arrow", "Left Bow Valve", "Left Bow Valve 1", "Left Bow Valve 2", "Left Down Elbow", "Left Down Elbow 1", "Left Pump", "Left Pump 1", "Left Rect Valve", "Left Rect Valve 1", "Left Rect Valve 2", "Left Tee", "Left Tee 1", "Left Up Elbow", "Left Up Elbow 1", "Less Or Equal To 0?", "Less Or Equal?", "Less Than 0?", "Less?", "Lexical Class", "Line Feed Constant", "List Directory", "Listbox", "Listbox 1", "Listbox Symbol Ring Constant", "Local Variable", "Lock Range", "Logarithm Base 10", "Logarithm Base 2", "Logarithm Base X", "Logical Shift", "Lowered Rounded Box", "MATLAB Script", "MakeAddr", "Mantissa & Exponent", "Match First String", "Match Pattern", "Match True/False String", "Max & Min", "Menu Refnum", "Menu Ring", "Menu Ring 1", "Menu-Popup Ring", "Merge Signals", "Meter", "Meter 1", "Molar Gas Constant (J/(mol K))", "Motion Resource", "Motion Resource 1", "Motion Resource Constant", "Motor", "Motor 1", "Move", "Multicolumn Listbox", "Multicolumn Listbox 1", "Multicolumn Listbox 2", "Multicolumn Listbox 3", "Multicolumn Listbox 4", "Multiple Selection Listbox", "Multiple Selection Listbox 1", "Multiple Selection Listbox 2", "Multiple Selection Listbox 3", "Multiple Selection Multicolumn Listbox", "Multiply", "Multiply Array Elements", "Natural Logarithm", "Natural Logarithm (Arg +1)", "Natural Logarithm Base", "Natural Logarithm Of 10", "Natural Logarithm Of 2", "Natural Logarithm Of Pi", "Negate", "Negative Infinity", "New Directory", "New File", "New VI", "New VI Object", "Not", "Not A Number/Path/Refnum?", "Not A Path Constant", "Not And", "Not Equal To 0?", "Not Equal?", "Not Exclusive Or", "Not Or", "Not a Refnum Constant", "Not a Tag", "Number To Boolean Array", "Number To Decimal String", "Number To Engineering String", "Number To Exponential String", "Number To Fractional String", "Number To Hexadecimal String", "Number To Octal String", "Numeric Constant", "Numeric Control", "Numeric Control 1", "Numeric Indicator", "Numeric Indicator 1", "OK Button", "OLE Variant", "Obtain Notifier", "Obtain Queue", "Occurrence Refnum", "Octal Digit?", "Octal String To Number", "Old VISA Open", "One Button Dialog", "Open Application Reference", "Open Device", "Open File", "Open File (New)", "Open Tank", "Open Tank 1", "Open VI Object Reference", "Open VI Reference", "Or", "Or Array Elements", "PPoll", "PPollConfig", "PPollUnconfig", "PassControl", "Path Constant", "Path To String", "Path Type", "Path to Array of Strings", "Pi", "Pi Divided By 2", "Pi Multiplied By 2", "Pick Line", "Pict Ring", "Pict Ring 1", "Picture", "PixMap", "PixMap (Do not touch it!!)", "Planck Constant (J/Hz)", "Platform Flat Square Button", "Plug-In Control", "Polar To Complex", "Positive Infinity", "Power Of 10", "Power Of 2", "Power Of X", "Pressure Tank", "Pressure Tank 1", "Preview Queue Element", "Printable?", "Property Node", "Pulldown Menu Ring", "Push Button", "Quit LabVIEW", "Quotient & Remainder", "Radio Buttons", "Raised Box", "Raised Box 1", "Raised Circle", "Raised Down Triangle", "Raised Frame", "Raised Left Triangle", "Raised Right Triangle", "Raised Rounded Box", "Raised Up Triangle", "Random Number (0-1)", "RcvRespMsg", "Re/Im To Complex", "Read Binary File", "Read Device", "Read File", "ReadStatus", "Receive", "ReceiveSetup", "Recessed Box", "Recessed Circle", "Recessed Down Triangle", "Recessed Frame", "Recessed Left Triangle", "Recessed Menu Ring", "Recessed Right Triangle", "Recessed Rounded Box", "Recessed Up Triangle", "Reciprocal", "Reciprocal Of Pi", "Reciprocal Of e", "Rectangular Stop Button", "Refnum to Path", "Refnum to Session", "Register Event Callback", "Register For Events", "Register Session", "Release Notifier", "Release Queue", "Replace Array Subset", "Replace Substring", "Request Deallocation", "ResetSys", "Reshape Array", "Reverse 1D Array", "Reverse String", "Right Arrow", "Right Bow Valve", "Right Bow Valve 1", "Right Bow Valve 2", "Right Down Elbow", "Right Down Elbow 1", "Right Pump", "Right Pump 1", "Right Rect Valve", "Right Rect Valve 1", "Right Rect Valve 2", "Right Tee", "Right Tee 1", "Right Up Elbow", "Right Up Elbow 1", "Ring Constant", "Rocker", "Rotary Feeder", "Rotate", "Rotate 1D Array", "Rotate Left With Carry", "Rotate Right With Carry", "Rotate String", "Round Button", "Round LED", "Round LED 1", "Round Light", "Round Push Button", "Round Push Button 2", "Round Radio Button", "Round Stop Button", "Round To +Infinity", "Round To -Infinity", "Round To Nearest", "Rydberg Constant (/m)", "Scale By Power Of 2", "Scan From File", "Scan From String", "Scan String For Tokens", "Scan Value", "Search 1D Array", "Search and Replace String", "Search/Split String", "Secant", "Seconds To Date/Time", "Seek", "Select", "Send", "Send Notification", "SendCmds", "SendDataBytes", "SendIFC", "SendLLO", "SendList", "SendSetup", "Session to Refnum", "Set Menu Item Info", "Set Occurrence", "Set Variant Attribute", "Set Waveform Attribute", "SetRWLS", "SetTimeOut", "Sign", "Simple Horizontal Slide", "Simple Numeric", "Simple Numeric 1", "Simple String", "Simple Vertical Slide", "Simulation Loop", "Sinc", "Sine", "Sine & Cosine", "Single Selection Listbox", "Size Handle", "Slide Switch", "Sort 1D Array", "Speed Of Light In Vacuum (m/sec)", "Split 1D Array", "Split Button", "Split Number", "Split Signals", "Spreadsheet String To Array", "Square Button", "Square LED", "Square LED 1", "Square Light", "Square Push Button", "Square Push Button 2", "Square Radio Button", "Square Root", "Stacked Sequence Structure", "Standard ListBox", "State Diagram", "Static VI Reference", "Stop", "Stop Button", "String Constant", "String Control", "String Control 1", "String Indicator", "String Indicator 1", "String Length", "String Subset", "String To Byte Array", "String To IP", "String To Path", "String to Tag", "Strip Path", "SubPanel", "SubPanel (Classic)", "Subtract", "Swap Bytes", "Swap Vector Element", "Swap Words", "TCP Close Connection", "TCP Create Listener", "TCP Flattened Read", "TCP Flattened Write", "TCP Flex Read", "TCP Flex Write", "TCP Network Connection Refnum", "TCP Open Connection", "TCP Read", "TCP Wait On Listener", "TCP Write", "Tab Constant", "Tab Control", "Tab Control 1", "Table", "Table 1", "Table 2", "Tag Attribute Ring", "Tag Constant", "Tag Control", "Tag Control 1", "Tag Indicator", "Tag Indicator 1", "Tag to String", "Tangent", "Tank", "Tank 1", "Temporary Directory", "TestSRQ", "TestSys", "Text & Pict Ring", "Text & Pict Ring 1", "Text Button", "Text Ring", "Text Ring 1", "Thermometer", "Thermometer 1", "Thick Chiseled Line", "Thick Line", "Thick Line with Arrow", "Thick Lowered Box", "Thin Chiseled Line", "Thin Line", "Thin Line with Arrow", "Threshold 1D Array", "Tick Count (ms)", "Time Stamp Constant", "Time Stamp Control", "Time Stamp Control 1", "Time Stamp Indicator", "Time Stamp Indicator 1", "Timed Loop", "To Byte Integer", "To Double Precision Complex", "To Double Precision Float", "To Extended Precision Complex", "To Extended Precision Float", "To Long Integer", "To Lower Case", "To More Generic Class", "To More Specific Class", "To OLE Variant", "To Quad Integer", "To Single Precision Complex", "To Single Precision Float", "To Time Stamp", "To Unsigned Byte Integer", "To Unsigned Long Integer", "To Unsigned Quad Integer", "To Unsigned Word Integer", "To Upper Case", "To Variant", "To Word Integer", "Traditional DAQ Channel", "Traditional DAQ Channel 1", "Traditional DAQ Channel Constant", "Transpose 2D Array", "Tree", "Trigger", "TriggerList", "Two Button Dialog", "Type Cast", "Type and Creator", "UDP Close", "UDP Multicast Open", "UDP Network Connection Refnum", "UDP Open", "UDP Read", "UDP Write", "Unbundle", "Unbundle By Name", "Unflatten From String", "Unflatten From XML", "Uniform Dbl Waveform", "Uniform Int16 Waveform", "Unregister For Events", "Unregister Session", "Up Arrow", "Up Bow Valve", "Up Bow Valve 1", "Up Bow Valve 2", "Up Rect Valve", "Up Rect Valve 1", "Up Rect Valve 2", "Up Tee", "Up Tee 1", "User Item", "VI Library", "VI Refnum", "VISA Assert Interrupt Signal", "VISA Assert Trigger", "VISA Assert Utility Signal", "VISA Clear", "VISA Close", "VISA Disable Event", "VISA Discard Events", "VISA Enable Event", "VISA Find Resource", "VISA Flush I/O Buffer", "VISA GPIB Command", "VISA GPIB Control ATN", "VISA GPIB Control REN", "VISA GPIB Pass Control", "VISA GPIB Send IFC", "VISA In 16", "VISA In 32", "VISA In 8", "VISA Lock", "VISA Map Address", "VISA Map Trigger", "VISA Memory Allocation", "VISA Memory Free", "VISA Move", "VISA Move In 16", "VISA Move In 32", "VISA Move In 8", "VISA Move Out 16", "VISA Move Out 32", "VISA Move Out 8", "VISA Open", "VISA Out 16", "VISA Out 32", "VISA Out 8", "VISA Peek 16", "VISA Peek 32", "VISA Peek 8", "VISA Poke 16", "VISA Poke 32", "VISA Poke 8", "VISA Read", "VISA Read STB", "VISA Read To File", "VISA Refnum to Session", "VISA Resource Name", "VISA Resource Name Constant", "VISA Set I/O Buffer Size", "VISA Status Description", "VISA USB Control In", "VISA USB Control Out", "VISA Unlock", "VISA Unmap Address", "VISA Unmap Trigger", "VISA VXI Cmd or Query", "VISA Wait on Event", "VISA Write", "VISA Write From File", "VISA resource name", "Variant", "Variant To Data", "Variant To Flattened String", "Vert Line", "Vert Pipe", "Vert Pipe 1", "Vert Rocker", "Vertical Fill Slide", "Vertical Fill Slide 1", "Vertical Graduated Bar", "Vertical Pointer Slide", "Vertical Pointer Slide 1", "Vertical Progress Bar", "Vertical Slide", "Vertical Slide Switch", "Vertical Slide Switch 1", "Vertical Smooth Box", "Vertical Switch", "Vertical Toggle Switch", "Vertical Toggle Switch 1", "Volume Info", "Wait (ms)", "Wait For Activity", "Wait For Front Panel Activity", "Wait Until Next ms Multiple", "Wait for GPIB RQS", "Wait on Notification", "Wait on Notification from Multiple", "Wait on Occurrence", "WaitSRQ", "Waveform Chart", "Waveform Chart 1", "Waveform Chart 2", "Waveform Graph", "Waveform Graph 1", "While Loop", "While Loop 1", "White Space?", "Write Device", "Write File", "XY Graph", "XY Graph 1", "Xmath Script"]
                      n244 = New VI Object(vi object class=w692, owner refnum=w691, style=w693, position/next to=w690, 8:w696) -> (object refnum=w689:refnum<vi>, 0:w695:errorcluster)  [unwired: 3 out]
                      n245 = property class="Path"(reference=w689, error in=w695, "Browse Button:Visible"=FALSE) -> (reference out=w687:refnum<vi>, error out=w694:errorcluster)
                    }
                    frame "Cluster" {
                      w702 = refnum<vi> refnum  # Boolean
